vi "Read Boolean Input.vi"(8 "error in (no error)":errorcluster, 10 "Boolean Input in":T1, 11 "Modbus in":refnum<class "Modbus.lvclass">) -> (0 "error out":errorcluster, 2 "Boolean value":bool, 3 "Modbus out":refnum<class "Modbus.lvclass">)   [LabVIEW 2026, in "Modbus.lvlib" / "Modbus.lvclass"]
uses:
  Modbus.lvclass
  Types/Boolean Data.ctl
  Types/Modbus Table.ctl
  Modbus.lvclass/Modbus.ctl
  <vilib>/ni/Modbus Library/API/Master/Modbus Master.lvclass
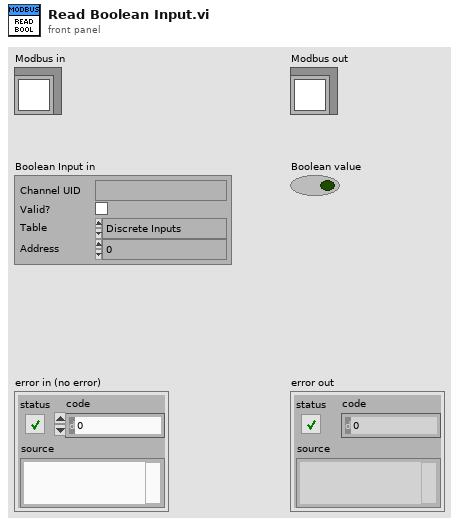
[diagram p1: front panel]
types:
  T1 = typedef "Modbus.lvlib/Modbus.lvclass/Boolean Data.ctl" = cluster{"Channel UID":string, "Valid?":bool, "Table":T2, "Address":i32}
  T2 = typedef "Modbus.lvlib/Modbus.lvclass/Modbus Table.ctl" = enum16{"Discrete Inputs", "Coils", "Input Registers", "Holding Registers"}
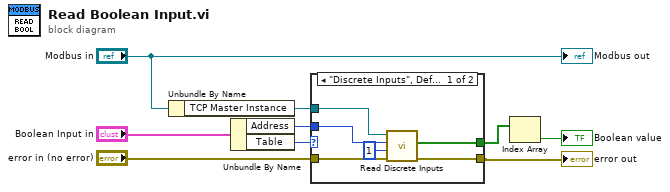
[diagram p0: block diagram]
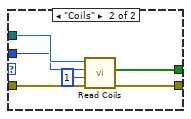
[diagram p2: hidden frame]
diagram:
  n1 = Unbundle By Name("Modbus in") -> ("TCP Master Instance"=w2:refnum<class "Modbus Master.lvclass">)
  n2 = Unbundle By Name("Boolean Input in") -> ("Address"=w4:i32, "Table"=w3:T2)
  n3 = case shown="\"Discrete Inputs\", Default" w3 {
    tunnel: w2 -> [w15 w21]
    tunnel: [w14 w20] -> w8
    tunnel: w4 -> [w13 w19]
    tunnel: [w12 w18] -> w1
    tunnel: "error in (no error)" -> [w10 w16]
    frame "Discrete Inputs", Default {
      n4 = call-dynamic "Read Discrete Inputs.vi"("error in"=w10, "number of inputs"=u16 1, "starting address"=w13, "Modbus master in"=w15) -> ("error out"=w14:errorcluster, "discrete inputs"=w12:bool[])  [unwired: 5 in, 1 out]
    }
    frame "Coils" {
      n5 = call-dynamic "Read Coils.vi"("error in"=w16, "number of inputs"=u16 1, "starting address"=w19, "Modbus master in"=w21) -> ("error out"=w20:errorcluster, "coils"=w18:bool[])  [unwired: 5 in, 1 out]
    }
  }
  "error out" <- w8
  n6 = Index Array(array=w1) -> (element=→"Boolean value":bool)  [unwired: 1 in]
  "Modbus out" <- "Modbus in"
